vi "OwnInterface20261013_MustOverride.vi"() -> ()   [LabVIEW 2024]
panel:
  out "error out":errorcluster caption="错误输出"
  in  "Save Class Path":path
  out "Actual":bool
  in  "Must Override":bool
  in  "Index":i32
  in  "Class Path":path
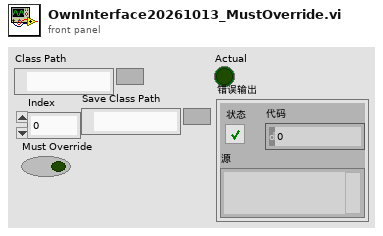
[diagram p1: front panel]
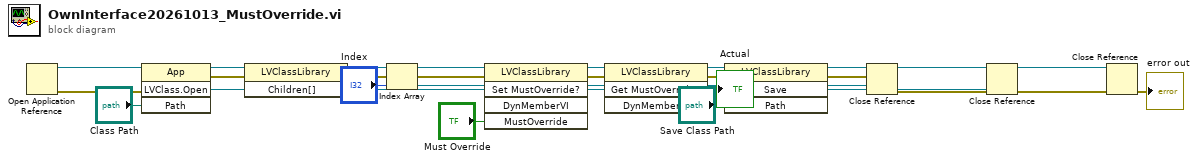
[diagram p0: block diagram]
diagram:
  n1 = Open Application Reference() -> (0:w16:errorcluster, 3:w18:refnum<vi>)  [unwired: 4 in]
  n2 = invoke class="App" method="LVClass.Open"(reference=w18, error in=w16, "Path"="Class Path") -> (error out=w14:errorcluster, "LVClass.Open"=w15:refnum<vi>)  [unwired: 1 in, 2 out]
  n3 = property class="LVClassLibrary"(reference=w15, error in=w14) -> (error out=w9:errorcluster, "Children[]"=w13:refnum<vi>[])  [unwired: 1 out]
  n4 = Index Array(array=w13, index="Index") -> (element=w11:refnum<vi>)
  n5 = invoke class="LVClassLibrary" method="Set MustOverride?"(reference=w15, error in=w9, "DynMemberVI"=w11, "MustOverride"="Must Override") -> (error out=w8:errorcluster)  [unwired: 1 in, 4 out]
  n6 = invoke class="LVClassLibrary" method="Get MustOverride?"(reference=w15, error in=w8, "DynMemberVI"=w11) -> (error out=w5:errorcluster, "GetMustOverride"=→"Actual":bool)  [unwired: 1 in, 2 out]
  n7 = invoke class="LVClassLibrary" method="Save"(reference=w15, error in=w5, "Path"="Save Class Path") -> (error out=w4:errorcluster)  [unwired: 1 in, 3 out]
  n8 = Close Reference(reference=w11, error in (no error)=w4) -> (error out=w3:errorcluster)
  n9 = Close Reference(reference=w15, error in (no error)=w3) -> (error out=w2:errorcluster)
  n10 = Close Reference(reference=w18, error in (no error)=w2) -> (error out=→"error out":errorcluster)
